vi "oled Error logger.vi"(8 "error in (no error)":errorcluster) -> (0 "error out":errorcluster)   [LabVIEW 2020]
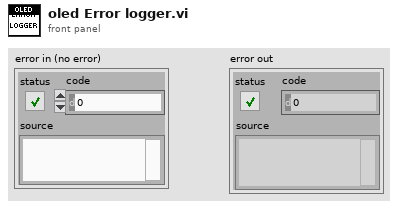
[diagram p1: front panel]
types:
  T1 = enum16{"open", "replace", "create", "open or create", "replace or create", "replace or create with confirmation"}
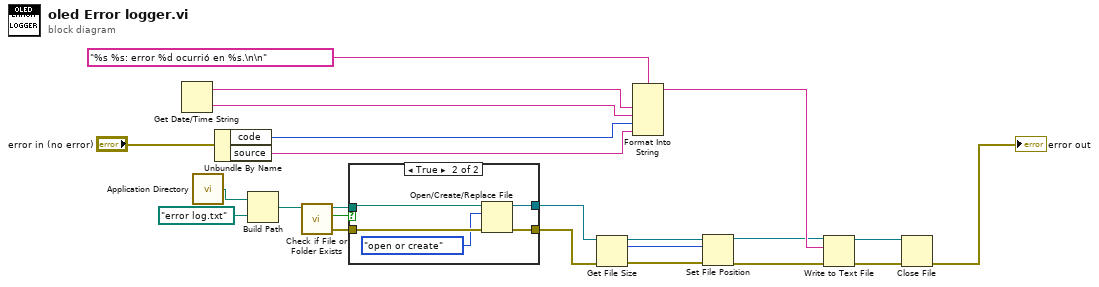
[diagram p0: block diagram]
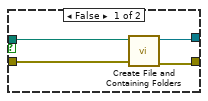
[diagram p2: hidden frame]
diagram:
  n1 = Get Date/Time String() -> (date string=w17:string, time string=w16:string)  [unwired: 3 in]
  n2 = call <vilib>:"Application Directory.vi"() -> ("Application Directory"=w20:path)
  n3 = Unbundle By Name("error in (no error)") -> ("code"=w14:i32, "source"=w13:string)
  n4 = Build Path(base path=w20, name or relative path=path "error log.txt") -> (appended path=w11:path)
  n5 = call <vilib>:"Check if File or Folder Exists.vi"("path"=w11) -> ("error out"=w8:errorcluster, "file or folder exists?"=w10:bool, "dup path"=w9:path)  [unwired: 8 in]
  n6 = case shown="True" w10 {
    tunnel: w9 -> [w27 w30]
    tunnel: w8 -> [w26 w32]
    tunnel: [w25 w31] -> w6
    tunnel: [w24 w29] -> w7
    frame False {
      n7 = call <vilib>:"Create File and Containing Folders.vi"("error in (no error)"=w26, "file path"=w27) -> ("error out"=w25:errorcluster, "refnum out"=w24:refnum<file>)  [unwired: 8 in]
    }
    frame True {
      n8 = Open/Create/Replace File(file path (use dialog)=w30, error in=w32, operation (0:open)=T1."open or create") -> (refnum out=w29:refnum<file>, error out=w31:errorcluster)  [unwired: 3 in, 1 out]
    }
  }
  n9 = Get File Size(file=w7, error in=w6) -> (refnum out=w4:refnum<file>, size (in bytes)=w3:i64, 0:w5:errorcluster)
  n10 = Format Into String(format string="%s %s: error %d ocurrió en %s.\n\n", w17, w16, w14, w13) -> (resulting string=w12:string)  [unwired: 2 in, 1 out]
  n11 = Set File Position(offset (in bytes) (0)=w3, refnum=w4, error in=w5) -> (refnum out=w2:refnum<file>, error out=w1:errorcluster)  [unwired: 1 in]
  n12 = Write to Text File(file (use dialog)=w2, text=w12, error in=w1) -> (refnum out=w23:refnum<file>, error out=w22:errorcluster)  [unwired: 1 in, 1 out]
  n13 = Close File(refnum=w23, error in=w22) -> (error out=→"error out":errorcluster)  [unwired: 1 out]
